vi "Get Array Value at Index - Known Type.vi"(6 "Get Value as JSON Tree? (F)":bool, 8 "error in (no error)":errorcluster, 10 "Index":i32, 11 "JSON Tree In (JSON Array)":variant) -> (0 "error out":errorcluster, 1 "is JSON Null?":bool, 2 "Value":variant, 3 "JSON Tree Out":variant, 4 "JSON Type":T2=enum."Unknown", 5 "JSON Compatible Type":T1=enum."Unknown")   [LabVIEW 2014, in "i3-json.lvlib"]
doc: "Returns the value at a given index from a JSON array"
uses:
  i3-json.lvlib
  JSON Types/JSON Type.ctl
  JSON Types/JSON Compatible Type.ctl
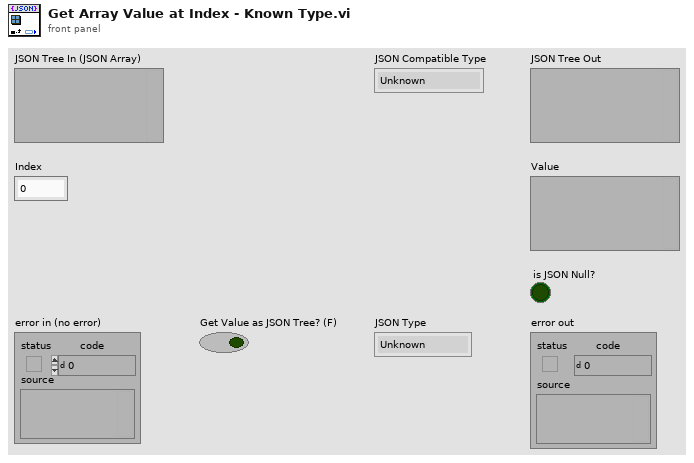
[diagram p1: front panel]
types:
  T1 = typedef "i3-json.lvlib/JSON Compatible Type.ctl" = enum16{"1D Double Array", "1D String Array", "1D Boolean Array", "Unknown"}
  T2 = typedef "i3-json.lvlib/JSON Type.ctl" = enum8{"JSON Compatible", "JSON Array", "JSON Object", "JSON Null", "Double", "String", "Boolean", "Unknown"}
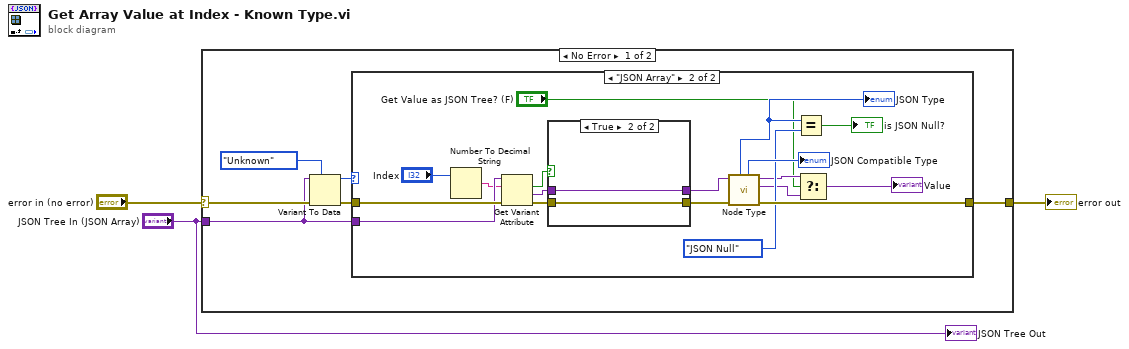
[diagram p0: block diagram]
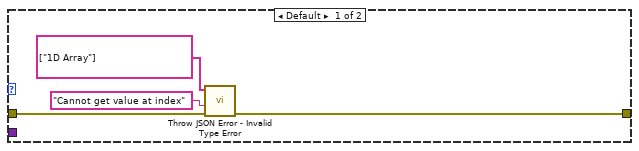
[diagram p2: hidden frame]
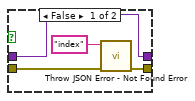
[diagram p3: hidden frame]
diagram:
  n1 = case shown="No Error" "error in (no error)" {
    selector: "error in (no error)" -> [w9 w38]
    tunnel: [w5 w38] -> w2
    tunnel: "JSON Tree In (JSON Array)" -> [w4 _]
    frame No Error {
      n2 = Variant To Data(error in=w9, type=JSON_Type."Unknown" ("JSON Type"), Variant=w4) -> (data=w6:T2, error out=w7:errorcluster)
      n3 = case shown="\"JSON Array\"" w6 {
        tunnel: w7 -> [w11 w31]
        tunnel: w4 -> [_ w29]
        tunnel: [w10 w27] -> w5
        frame Default {
          n4 = call "Throw JSON Error - Invalid Type Error.vi"("error in (no error)"=w11, "additional info"="Cannot get value at index", "Valid Types"=string[] ["1D Array"]) -> ("error out"=w10:errorcluster)  [unwired: 8 in]
        }
        frame "JSON Array" {
          n5 = Number To Decimal String(number="Index") -> (decimal integer string=w28:string)  [unwired: 1 in]
          n6 = Get Variant Attribute(Variant=w29, name=w28, error in=w31) -> (found=w21:bool, value=w23:variant, error out=w22:errorcluster)  [unwired: 1 in, 1 out]
          n7 = case shown="True" w21 {
            tunnel: w22 -> [w33 w37]
            tunnel: [w32 w37] -> w25
            tunnel: w23 -> [w35 w36]
            tunnel: [w35 w36] -> w24
            frame False {
              n8 = call "Throw JSON Error - Not Found Error.vi"("error in (no error)"=w33, "item type"="index") -> ("error out"=w32:errorcluster)  [unwired: 9 in]
            }
            frame True {
            }
          }
          n9 = call "Node Type.vi"("error in (no error)"=w25, "JSON Tree In"=w24) -> ("error out"=w27:errorcluster, "Value"=w15:variant, "JSON Tree Out"=w16:variant, "JSON Compatible Type"=→"JSON Compatible Type":T1, "JSON Type"=w19:T2)  [unwired: 5 in]
          "JSON Type" <- w19
          n10 = Equal?(x=w19, y=JSON_Type."JSON Null") -> (x = y?=→"is JSON Null?":bool)
          n11 = Select(t=w16, s="Get Value as JSON Tree? (F)", f=w15) -> (s? t:f=→"Value":variant)
        }
      }
    }
    frame Error {
    }
  }
  "error out" <- w2
  "JSON Tree Out" <- "JSON Tree In (JSON Array)"
